vi "GAP_AcquireImages.vi"() -> ()   [LabVIEW 2020]
uses:
  Control 2.ctl
  <vilib>/vision/driver/IMAQdx.llb/IMAQdx Buffer Number Mode.ctl
  <vilib>/vision/driver/NI_Vision_Acquisition_Software.lvlib
  <resource>/objmgr/imaqdx.rc
  <vilib>/vision/NI_Vision_Development_Module.lvlib
panel:
  in  "Save image":T1
  out "Original Image":T2(plugin-control)
  in  "Image Type":T3 items=["Grayscale (U8)", "Grayscale (I16)", "Grayscale (SGL)", "Complex (CSG)", "RGB (U32)", "HSL (U32)", "RGB (U64)", "Grayscale (U16)"]
  out "Frame rate":dbl
  in  "Stop image acquisition":bool
  in  "Stop Button":bool
  in  "Start acquisition":bool
  out "Line Profile":cluster{"x0":sgl, "dx":sgl, "Pixels Line":sgl[]}(graph)
  in  "Percent of Images Reserved by Driver":dbl=50.0
  in  "Overwrite Mode":u16(ring) items=["Get Oldest"=0, "Fail"=2, "Get Newest"=3]
  in  "Camera Name":refnum<k21> caption="IMAQdx Session"
  out "Grayscale Image":T2(plugin-control)
  out "Acquired imgs":u32
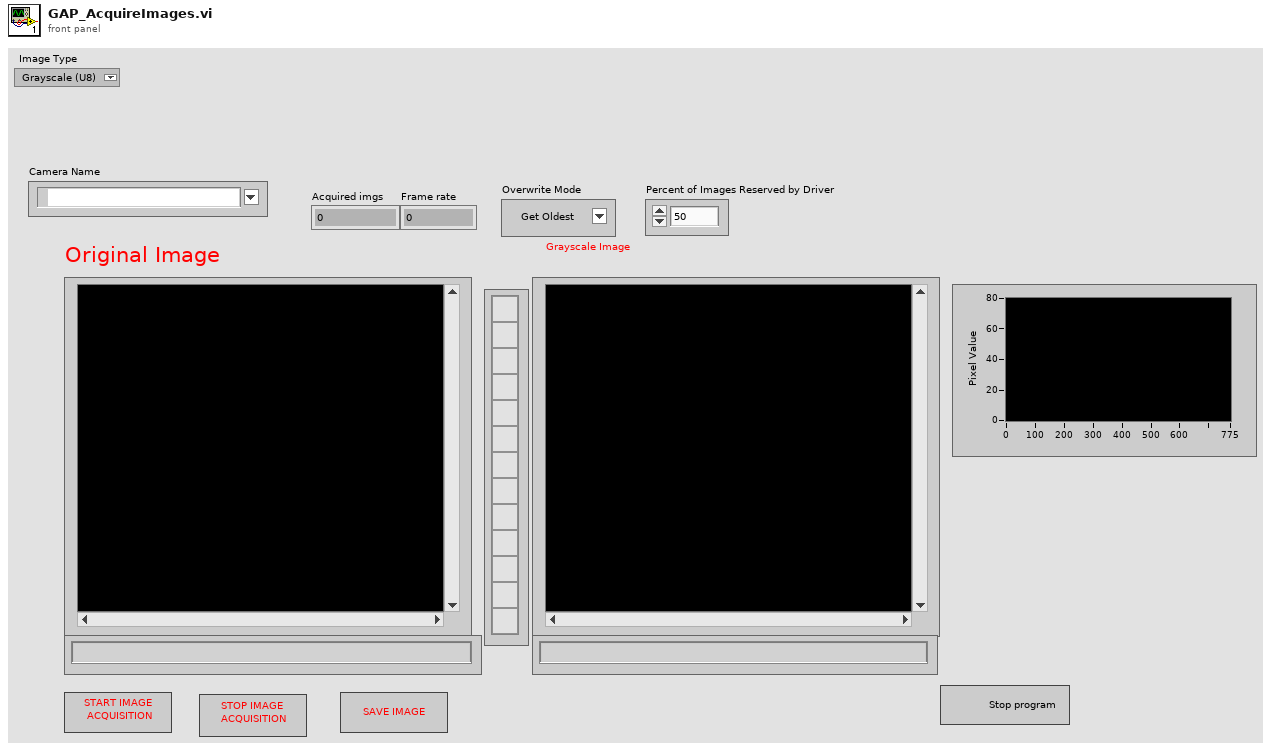
[diagram p1: front panel]
types:
  T1 = typedef "Control 2.ctl" = bool
  T2 = typedef "IMAQ Image.ctl" = refnum<image>
  T3 = typedef "Image Type" = u32
  T4 = typedef "NI_Vision_Acquisition_Software.lvlib/IMAQdx Buffer Number Mode.ctl" = enum32{"Next", "Last", "Buffer Number", "Every", "Last New"}
  T5 = typedef "IMAQdx.ctl" = refnum<k21>
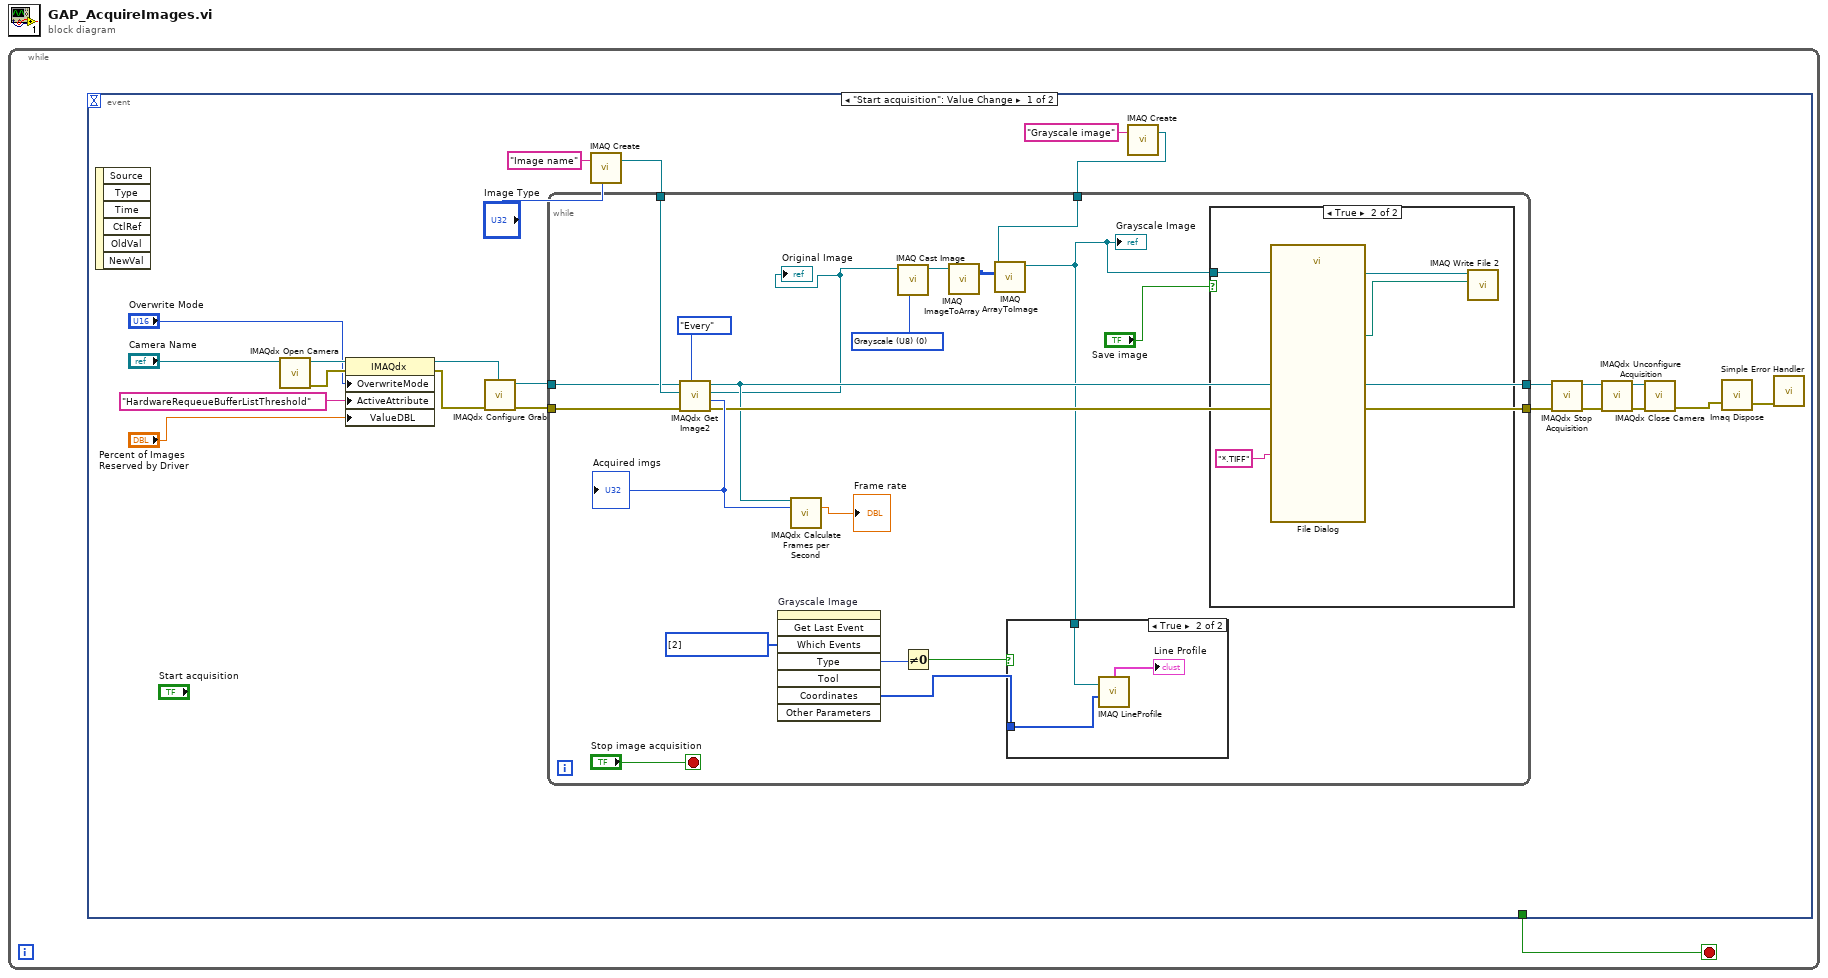
[diagram p0: block diagram]
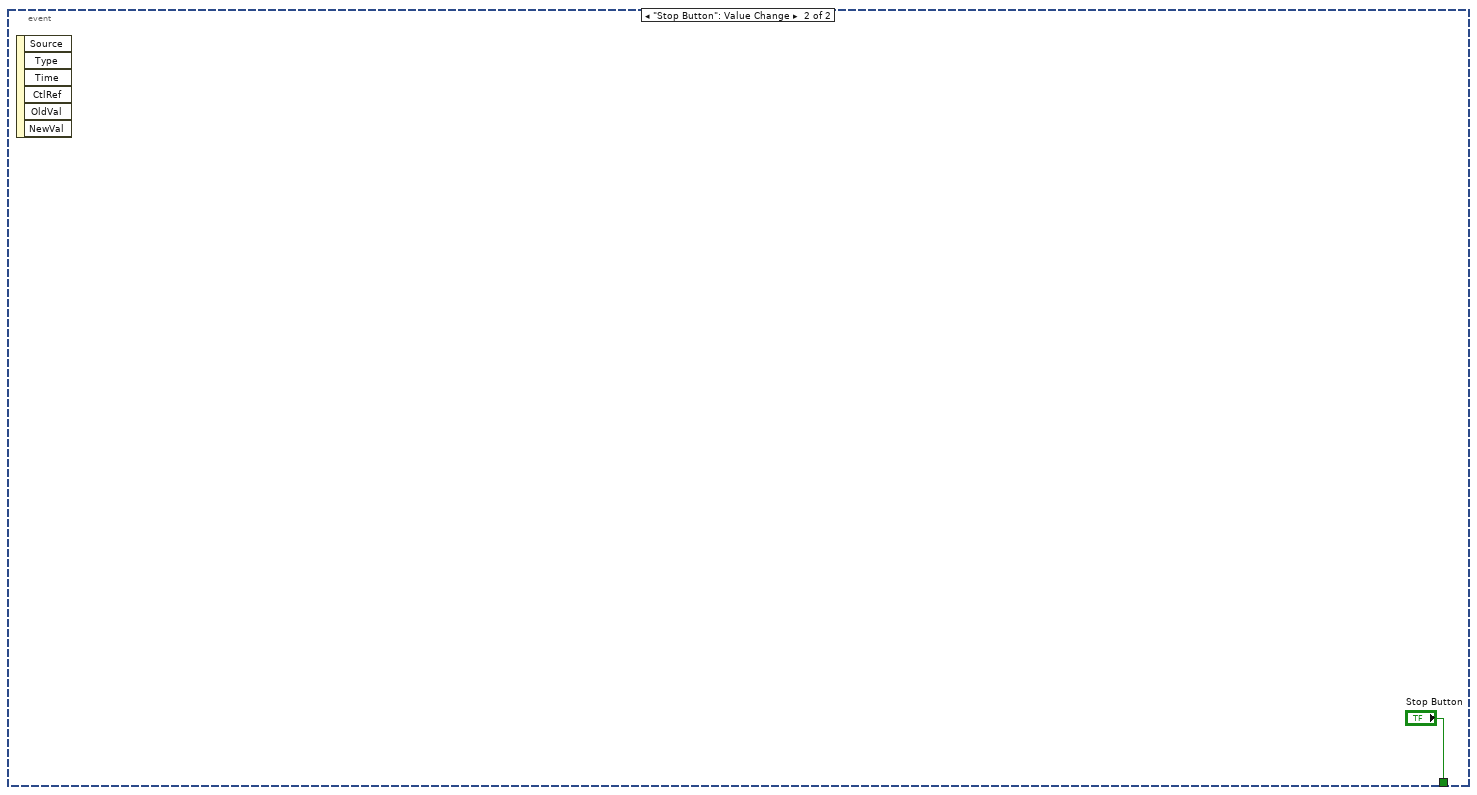
[diagram p4: hidden frame]
diagram:
  n1 = while {
    stop <- w1 stop-if-true
    n2 = event shown="[0] \"Start acquisition\": Value Change" {
      selector: _ -> [_ _]
      dyn-events: _ -> [_ _]
      timeout: _ -> [_ _]
      tunnel: [_ "Stop Button"] -> w1
      event "Start acquisition": Value Change {
        n3 = event-data() -> ()  [unwired: 1 in, 6 out]
        n4 = call <vilib>:"IMAQdx Open Camera.vi"("Session In"="Camera Name") -> ("error out"=w21:errorcluster, "Session Out"=w22:T5)  [unwired: 2 in, 7 out]
        n5 = property class="IMAQdx"(reference=w22, error in=w21, "OverwriteMode"="Overwrite Mode", "ActiveAttribute"="HardwareRequeueBufferListThreshold", "ValueDBL"="Percent of Images Reserved by Driver") -> (reference out=w17:T5, error out=w18:errorcluster)
        n6 = call <vilib>:"IMAQdx Configure Grab.vi"("error in"=w18, "Session In"=w17) -> ("error out"=w15:errorcluster, "Session Out"=w16:T5)  [unwired: 8 in]
        n7 = call "IMAQ Create"("Image Name"="Image name", "Image Type"="Image Type") -> ("New Image"=w13:T2)  [unwired: 2 in, 2 out]
        n8 = call "IMAQ Create"("Image Name"="Grayscale image") -> ("New Image"=w2:T2)  [unwired: 3 in, 2 out]
        n9 = while {
          tunnel: w13 -> [w43]
          tunnel: w16 -> [w41]
          tunnel: w15 -> [w40]
          tunnel: [w39] -> w6
          tunnel: [w38] -> w5
          tunnel: w2 -> [w28]
          stop <- "Stop image acquisition" stop-if-true
          w31 = T3 0 items=["Grayscale (U8)", "Grayscale (I16)", "Grayscale (SGL)", "Complex (CSG)", "RGB (U32)", "HSL (U32)", "RGB (U64)", "Grayscale (U16)"] ("Image Type")
          w37 = i32[] [2] items=["No Event"=0, "Click Event"=1, "Draw Event"=2, "Size Event"=4, "Scroll Event"=5, "Double Click Event"=8] ("Which Events")
          n10 = call <vilib>:"IMAQdx Get Image2.vi"("Buffer Number Mode (Next)"=IMAQdx_Buffer_Number_Mode."Every", "error in"=w40, "Image In"=w43, "Session In"=w41) -> ("error out"=w39:errorcluster, "Buffer Number Out"=w44:u32, "Image Out"=w27:T2, "Session Out"=w38:T5)  [unwired: 4 in]
          "Acquired imgs" <- w44
          "Original Image" <- w27
          n11 = invoke on="Grayscale Image" class="ImageControl" method="Get Last Event"("Which Events"=w37) -> ("Type"=w36:i32, "Coordinates"=w34:i32[])  [unwired: 7 in, 6 out]
          n12 = call <vilib>:"IMAQdx Calculate Frames per Second.vi"("Session In"=w38, "Buffer Number"=w44) -> ("Acquired Frames per Second"=→"Frame rate":dbl)  [unwired: 7 in, 6 out]
          n13 = call "IMAQ Cast Image"("Image Type"=w31, "Image Src"=w27) -> ("Image Dst Out"=w30:T2)  [unwired: 4 in, 5 out]
          n14 = Not Equal To 0?(x=w36) -> (x != 0?=w35:bool)
          n15 = call "IMAQ ImageToArray"("Image"=w30) -> ("Image Pixels (U8)"=w29:u8[][])  [unwired: 3 in, 4 out]
          n16 = call "IMAQ ArrayToImage"("Image Pixels (U8)"=w29, "Image"=w28) -> ("Image Out"=w25:T2)  [unwired: 8 in, 1 out]
          "Grayscale Image" <- w25
          n17 = case shown="True" w35 {
            tunnel: w34 -> [_ w49]
            tunnel: w25 -> [_ w48]
            frame False {
            }
            frame True {
              n18 = call "IMAQ LineProfile"("Line Coordinates"=w49, "Image"=w48) -> ("Line Graph"=→"Line Profile":cluster{"x0":sgl, "dx":sgl, "Pixels Line":sgl[]})  [unwired: 3 in, 3 out]
            }
          }
          n19 = case shown="True" "Save image" {
            tunnel: w25 -> [_ w47]
            frame False {
            }
            frame True {
              n20 = call "File Dialog"("pattern (all files)"="*.TIFF" ("pattern label")) -> ("selected path"=w46:path)  [unwired: 11 in, 3 out]
              n21 = call-poly "IMAQ Write File 2"("File Path"=w46, "Image"=w47) -> ()  [unwired: 8 in, 2 out]
            }
          }
        }
        n22 = call <vilib>:"IMAQdx Stop Acquisition.vi"("error in"=w6, "Session In"=w5) -> ("error out"=w8:errorcluster, "Session Out"=w9:T5)  [unwired: 8 out]
        n23 = call <vilib>:"IMAQdx Unconfigure Acquisition.vi"("error in"=w8, "Session In"=w9) -> ("error out"=w10:errorcluster, "Session Out"=w11:T5)  [unwired: 8 out]
        n24 = call <vilib>:"IMAQdx Close Camera.vi"("error in"=w10, "Session In"=w11) -> ("error out"=w7:errorcluster)  [unwired: 9 out]
        n25 = call "Imaq Dispose"("error in (no error)"=w7) -> ("error out"=w12:errorcluster)  [unwired: 5 in]
        n26 = call <vilib>:"Simple Error Handler.vi"("error in (no error)"=w12) -> ()  [unwired: 4 in, 5 out]
      }
      event "Stop Button": Value Change {
        n27 = event-data() -> ()  [unwired: 1 in, 6 out]
      }
    }
  }
